vi "set ACLR Tx Channel Count.vi"(8 "error in (no error)":errorcluster, 10 "Tx Channel Count":i32=1 min=1, 11 "FSV-40N in":refnum<class "FSV-40N.lvclass">) -> (0 "error out":errorcluster, 3 "FSV-40N out":refnum<class "FSV-40N.lvclass">)   [LabVIEW 2023, in "Spectrum Analyzer.lvlib" / "FSV-40N.lvclass"]
uses:
  FSV-40N.lvclass
  FSV-40N.lvclass/FSV-40N.ctl
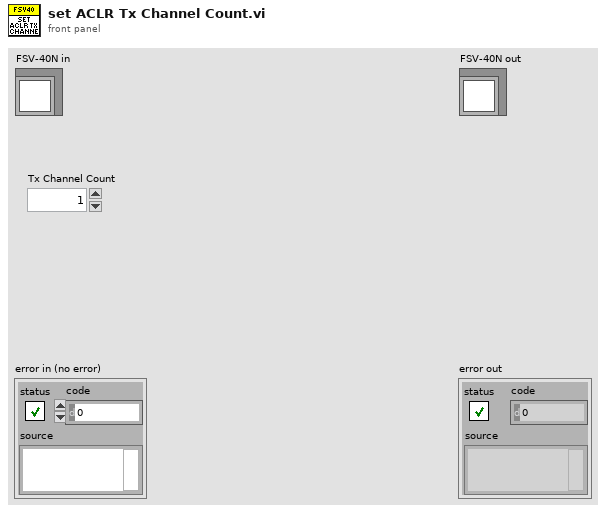
[diagram p1: front panel]
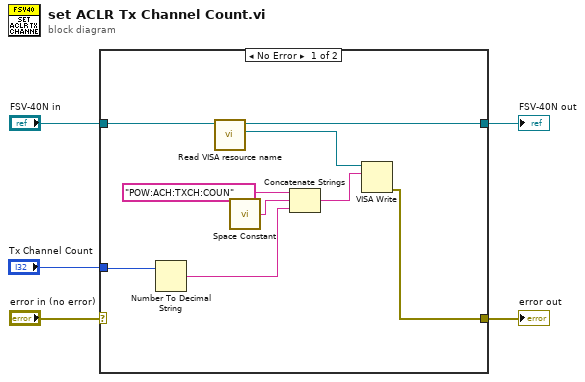
[diagram p0: block diagram]
diagram:
  n1 = case shown="No Error" "error in (no error)" {
    selector: "error in (no error)" -> [_ w15]
    tunnel: "FSV-40N in" -> [w14 w16]
    tunnel: [w7 w16] -> w3
    tunnel: [w6 w15] -> w2
    tunnel: "Tx Channel Count" -> [w11 _]
    frame No Error {
      n2 = Number To Decimal String(number=w11) -> (decimal integer string=w10:string)  [unwired: 1 in]
      n3 = call "Read VISA resource name.vi"("FSV-40N in"=w14) -> ("VISA resource name"=w9:refnum<visa-resource-name>, "FSV-40N out"=w7:refnum<class "FSV-40N.lvclass">)  [unwired: 8 in, 1 out]
      n4 = call <vilib>:"Space Constant.vi"() -> ("String"=w12:string)
      n5 = Concatenate Strings("POW:ACH:TXCH:COUN" ("string"), w12, w10) -> (w8:string)
      n6 = VISA Write(VISA resource name=w9, write buffer=w8) -> (error out=w6:errorcluster)  [unwired: 1 in, 2 out]
    }
    frame Error {
    }
  }
  "error out" <- w2
  "FSV-40N out" <- w3
